vi "VIH UI - Tree Value Changed.vi"(7 "SubPanel":refnum<vi>, 8 "error in":errorcluster, 11 "Project Tree":T1) -> (0 "error out":errorcluster, 1 "Item Title":string, 2 "Item Icon":picture, 3 "dup Tree Refnum":T1)   [LabVIEW 2014]
doc: "::: VI Helpeks :::\nCopyright (c) 2000-2026 Konstantin Shifershteyn. All rights reserved."
uses:
  VIH Project Tree Typedef - Tree Refnum.ctl
panel:
  # "VI Helpeks\nCopyright (c) 2012-2026 Konstantin Shifershteyn"
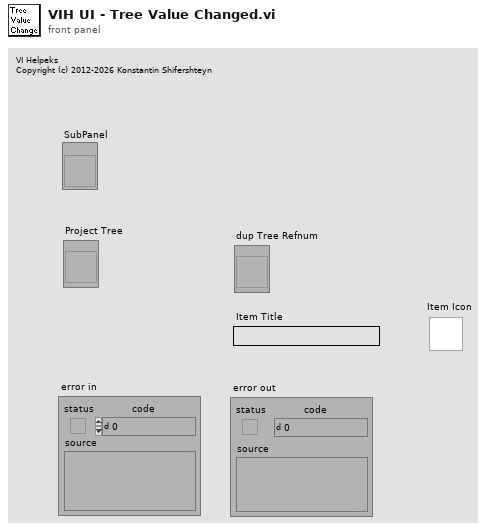
[diagram p1: front panel]
types:
  T1 = typedef "VIH Project Tree Typedef - Tree Refnum.ctl" = refnum<vi>
  T2 = typedef "VIH Project Tree Typedef - Tree Item Type.ctl" = enum32{"<Invalid>", "Project", "Proj Files", "Proj Rules", "File Group", "Rule Group", "Any File", "LV Func", ".mnu", ".mnu (dyn)", ".vi", ".vi (dyn)", ".vit", ".vit (dyn)", ".ctl", ".ctl (dyn)", ".ctt", ".ctt (dyn)", "polyVI", "polyVI (dyn)", "expVI", "expVI (dyn)", "HTML", "PolyVI Inst"}
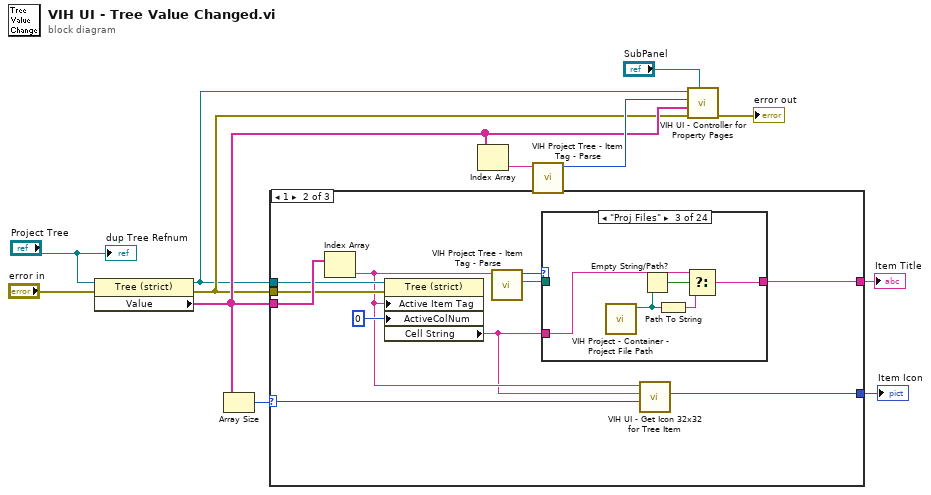
[diagram p0: block diagram]
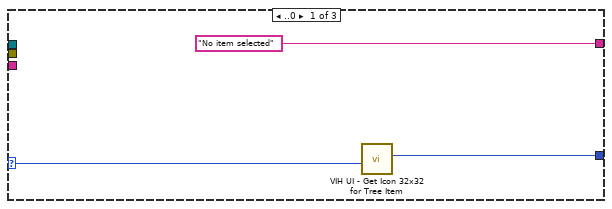
[diagram p2: hidden frame]
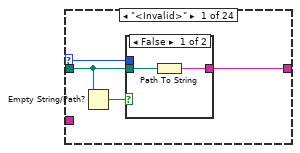
[diagram p3: hidden frame]
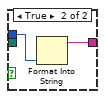
[diagram p4: hidden frame]
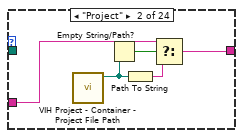
[diagram p5: hidden frame]
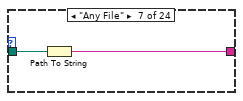
[diagram p9: hidden frame]
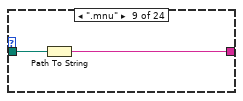
[diagram p11: hidden frame]
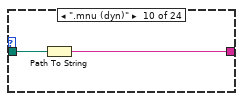
[diagram p12: hidden frame]
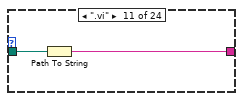
[diagram p13: hidden frame]
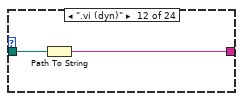
[diagram p14: hidden frame]
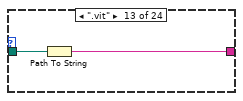
[diagram p15: hidden frame]
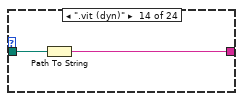
[diagram p16: hidden frame]
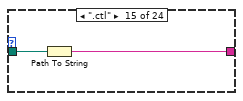
[diagram p17: hidden frame]
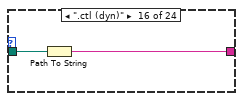
[diagram p18: hidden frame]
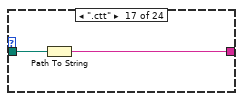
[diagram p19: hidden frame]
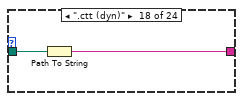
[diagram p20: hidden frame]
diagram:
  n1 = property class="Tree (strict)"(reference="Project Tree", error in="error in") -> (reference out=w2:T1, error out=w4:errorcluster, "Value"=w9:string[])
  n2 = Array Size(array=w9) -> (size(s)=w10:i32)
  n3 = case shown="1" w10 {
    selector: w10 -> [w13 w16 w94]
    tunnel: w9 -> [_ w26 w85]
    tunnel: ["No item selected" ("Cell String") w24 w96] -> w5
    tunnel: w2 -> [_ w21 w86]
    tunnel: w4 -> [_ w20 w84]
    tunnel: [w14 w17 w95] -> w1
    frame ..0 {
      n4 = call "VIH UI - Get Icon 32x32 for Tree Item.vi"("# Items (1)"=w13) -> ("Item Icon"=w14:picture)  [unwired: 9 in, 1 out]
    }
    frame 1 {
      n5 = Index Array(array=w26) -> (element=w19:string)  [unwired: 1 in]
      n6 = property on="Property Node" class="Tree (strict)"(reference=w21, error in=w20, "Active Item Tag"=w19, "ActiveColNum"=0 ("Active Cell:Active Column Number")) -> ("Cell String"=w18:string)  [unwired: 2 out]
      n7 = call "VIH Project Tree - Item Tag - Parse.vi"("Tree Item Tag"=w19) -> ("Item File Path"=w25:path, "Item Type"=w22:T2)  [unwired: 8 in, 1 out]
      n8 = case shown="\"Proj Files\"" w22 {
        selector: w22 -> [w30 _ _ _ _ _ _ _ _ _ _ _ _ _ _ _ _ _ _ _ _ _ _ _]
        tunnel: w25 -> [w27 _ _ _ _ _ w49 _ w52 w54 w56 w58 w60 w62 w64 w66 w68 w70 w72 w74 w76 w78 w80 w82]
        tunnel: [w29 w35 w40 w45 w46 w47 w48 w50 w51 w53 w55 w57 w59 w61 w63 w65 w67 w69 w71 w73 w75 w77 w79 w81] -> w24
        tunnel: w18 -> [_ w38 w43 w45 w46 w47 _ w50 _ _ _ _ _ _ _ _ _ _ _ _ _ _ _ _]
        frame "<Invalid>" {
          n9 = Empty String/Path?(string/path=w27) -> (empty?=w28:bool)
          n10 = case shown="False" w28 {
            tunnel: w30 -> [_ w34]
            tunnel: [w32 w33] -> w29
            tunnel: w27 -> [w31 _]
            frame False {
              n11 = Path To String(path=w31) -> (string=w32:string)
            }
            frame True {
              n12 = Format Into String(w34) -> (resulting string=w33:string)  [unwired: 3 in, 1 out]
            }
          }
        }
        frame "Project" {
          n13 = call "VIH Project - Container - Project File Path.vi"() -> ("Project File Path"=w39:path)  [unwired: 9 in, 2 out]
          n14 = Empty String/Path?(string/path=w39) -> (empty?=w36:bool)
          n15 = Path To String(path=w39) -> (string=w37:string)
          n16 = Select(t=w38, s=w36, f=w37) -> (s? t:f=w35:string)
        }
        frame "Proj Files" {
          n17 = call "VIH Project - Container - Project File Path.vi"() -> ("Project File Path"=w44:path)  [unwired: 9 in, 2 out]
          n18 = Empty String/Path?(string/path=w44) -> (empty?=w41:bool)
          n19 = Path To String(path=w44) -> (string=w42:string)
          n20 = Select(t=w43, s=w41, f=w42) -> (s? t:f=w40:string)
        }
        frame "Proj Rules" {
        }
        frame "File Group" {
        }
        frame "Rule Group" {
        }
        frame "Any File" {
          n21 = Path To String(path=w49) -> (string=w48:string)
        }
        frame "LV Func" {
        }
        frame ".mnu" {
          n22 = Path To String(path=w52) -> (string=w51:string)
        }
        frame ".mnu (dyn)" {
          n23 = Path To String(path=w54) -> (string=w53:string)
        }
        frame ".vi" {
          n24 = Path To String(path=w56) -> (string=w55:string)
        }
        frame ".vi (dyn)" {
          n25 = Path To String(path=w58) -> (string=w57:string)
        }
        frame ".vit" {
          n26 = Path To String(path=w60) -> (string=w59:string)
        }
        frame ".vit (dyn)" {
          n27 = Path To String(path=w62) -> (string=w61:string)
        }
        frame ".ctl" {
          n28 = Path To String(path=w64) -> (string=w63:string)
        }
        frame ".ctl (dyn)" {
          n29 = Path To String(path=w66) -> (string=w65:string)
        }
        frame ".ctt" {
          n30 = Path To String(path=w68) -> (string=w67:string)
        }
        frame ".ctt (dyn)" {
          n31 = Path To String(path=w70) -> (string=w69:string)
        }
        frame "polyVI" {
          n32 = Path To String(path=w72) -> (string=w71:string)
        }
        frame "polyVI (dyn)" {
          n33 = Path To String(path=w74) -> (string=w73:string)
        }
        frame "expVI" {
          n34 = Path To String(path=w76) -> (string=w75:string)
        }
        frame "expVI (dyn)" {
          n35 = Path To String(path=w78) -> (string=w77:string)
        }
        frame "HTML" {
          n36 = Path To String(path=w80) -> (string=w79:string)
        }
        frame "PolyVI Inst" {
          n37 = Path To String(path=w82) -> (string=w81:string)
        }
      }
      n38 = call "VIH UI - Get Icon 32x32 for Tree Item.vi"("# Items (1)"=w16, "Item Name"=w18, "Tree Item Tag"=w19) -> ("Item Icon"=w17:picture)  [unwired: 7 in, 1 out]
    }
    frame 2.. {
      n39 = for {
        tunnel: w85 -> [w112] mode=indexing
        tunnel: [w111] -> w97 mode=indexing
        n40 = call "VIH Project Tree - Item Tag - Parse.vi"("Tree Item Tag"=w112) -> ("Item File Path"=w111:path)  [unwired: 8 in, 2 out]
      }
      n41 = call "VIH Utility - FILE - Remove Duplicated Paths from 1D Array.vi"("Array in"=w97) -> ("Array out"=w91:path[])  [unwired: 9 in, 1 out]
      n42 = Array Size(array=w91) -> (size(s)=w93:i32)
      n43 = Index Array(array=w91) -> (element=w87:path)  [unwired: 1 in]
      n44 = Empty String/Path?(string/path=w87) -> (empty?=w89:bool)
      n45 = Equal?(x=1, y=w93) -> (x = y?=w90:bool)
      n46 = Not(x=w89) -> (.not. x?=w83:bool)
      n47 = And(x=w90, y=w83) -> (x .and. y?=w88:bool)
      n48 = case shown="False" w88 {
        tunnel: ["Multiple selection" w108] -> w96
        tunnel: [w100 w110] -> w95
        tunnel: w94 -> [w99 _]
        tunnel: w87 -> [_ w109]
        tunnel: w86 -> [_ w106]
        tunnel: w85 -> [_ w105]
        tunnel: w84 -> [_ w101]
        frame False {
          (unwired) "Multiple items selected"
          n49 = call "VIH UI - Get Icon 32x32 for Tree Item.vi"("# Items (1)"=w99) -> ("Item Icon"=w100:picture)  [unwired: 9 in, 1 out]
        }
        frame True {
          n50 = Index Array(array=w105) -> (element=w104:string)  [unwired: 1 in]
          n51 = Path To String(path=w109) -> (string=w108:string)
          n52 = property on="Property Node" class="Tree (strict)"(reference=w106, error in=w101, "Active Item Tag"=w104, "ActiveColNum"=0 ("Active Cell:Active Column Number")) -> ("Cell String"=w103:string)  [unwired: 2 out]
          n53 = call "VIH UI - Get Icon 32x32 for Tree Item.vi"("# Items (1)"=1, "Item Name"=w103, "Tree Item Tag"=w104) -> ("Item Icon"=w110:picture)  [unwired: 7 in, 1 out]
        }
      }
    }
  }
  "Item Title" <- w5
  "Item Icon" <- w1
  n54 = Index Array(array=w9) -> (element=w11:string)  [unwired: 1 in]
  n55 = call "VIH Project Tree - Item Tag - Parse.vi"("Tree Item Tag"=w11) -> ("Item Type"=w12:T2)  [unwired: 8 in, 2 out]
  n56 = call "VIH UI - Controller for Property Pages.vi"("SubPanel"="SubPanel", "error in"=w4, "Params"=w9, "Item Type"=w12, "Project Tree"=w2) -> ("error out"=→"error out":errorcluster)  [unwired: 5 in, 1 out]
  "dup Tree Refnum" <- "Project Tree"
